vi "SPARK Get Closed Loop Status.vi"   [LabVIEW 2027]
doc: "Get the status of the closed loop controller of the SPARK."
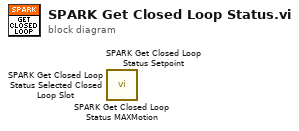
[diagram p0: block diagram]
diagram:
  n1 = call <vilib>:"SPARK Get Closed Loop Status MAXMotion.vi"() -> ()  [unwired: 7 in, 5 out]
  n2 = call <vilib>:"SPARK Get Closed Loop Status Setpoint.vi"() -> ()  [unwired: 7 in, 5 out]
  n3 = call <vilib>:"SPARK Get Closed Loop Status Selected Closed Loop Slot.vi"() -> ()  [unwired: 8 in, 4 out]
